vi "RemoteVI Hover Decision.vi"(0 "menus":T2(array[cluster]), 5 "state":T1, 7 "now":u32) -> (4 "navigate?":bool, 6 "dwell?":bool, 8 "parent?":bool, 10 "k":i32=-1)   [LabVIEW 2020, in "RemoteVI.lvlib"]
doc: "Decides what the remote pointer (state.x, state.y) asks of the open LabVIEW menus (RemoteVI List Menus.vi, deepest first): k is the menu under the pointer (RemoteVI Point On Popup.vi). navigate? - it is over the DEEPEST menu at a position not applied yet; dwell? - it has stayed on the highlighted item of the deepest menu (state.menu, state.hit) for 400 ms since row since and VK_RIGHT has not been posted for it; parent? - it is over a parent of open submenus at a position not applied yet. All three are FALSE when the pointer is over no menu, or when the deepest popup takes no keys (state.plain: colour picker, line width popup - neither it nor its parents can be driven with keys then). Pure."
uses:
  RemoteVI.lvlib
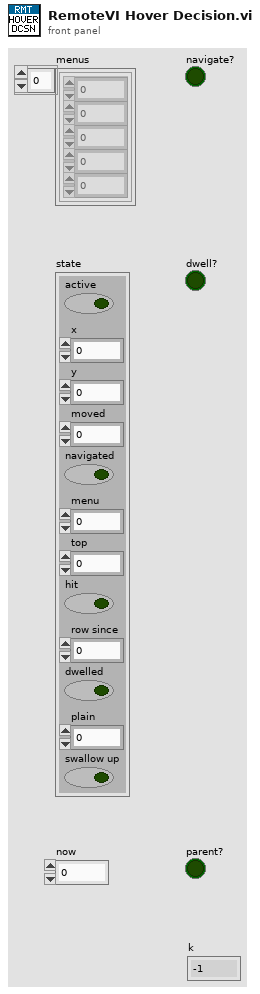
[diagram p1: front panel]
types:
  T1 = cluster{"active":bool, "x":i32, "y":i32, "moved":u32, "navigated":bool, "menu":u64, "top":i32, "hit":bool, "row since":u32, "dwelled":bool, "plain":u64, "swallow up":bool}
  T2 = cluster{"hwnd":u64, "x":i32, "y":i32, "w":i32, "h":i32}[]
  T3 = cluster{"hwnd":u64, "x":i32, "y":i32, "w":i32, "h":i32}
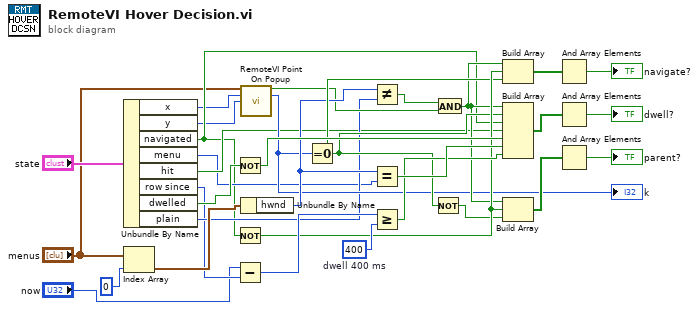
[diagram p0: block diagram]
diagram:
  w27 = u32 400  # dwell 400 ms
  n1 = Unbundle By Name("state") -> ("x"=w4:i32, "y"=w5:i32, "navigated"=w6:bool, "menu"=w7:u64, "hit"=w8:bool, "row since"=w9:u32, "dwelled"=w10:bool, "plain"=w11:u64)
  n2 = Index Array(array="menus", index=0) -> (element=w15:T3)
  n3 = Not(x=w10) -> (.not. x?=w30:bool)
  n4 = Not(x=w6) -> (.not. x?=w21:bool)
  n5 = Subtract(x="now", y=w9) -> (x-y=w26:u32)
  n6 = call "RemoteVI Point On Popup.vi"("windows"="menus", "x"=w4, "y"=w5) -> ("on popup?"=w12:bool, "index"=w13:i32)  [unwired: 11 in]
  "k" <- w13
  n7 = Unbundle By Name(w15) -> ("hwnd"=w16:u64)
  n8 = Equal To 0?(x=w13) -> (x = 0?=w19:bool)
  n9 = Not Equal?(x=w16, y=w11) -> (x != y?=w17:bool)
  n10 = Equal?(x=w16, y=w7) -> (x = y?=w29:bool)
  n11 = Greater Or Equal?(x=w26, y=w27) -> (x >= y?=w28:bool)
  n12 = Not(x=w19) -> (.not. x?=w20:bool)
  n13 = And(x=w17, y=w12) -> (x .and. y?=w18:bool)
  n14 = Build Array(w18, w21, w19) -> (w22:bool[])
  n15 = Build Array(w18, w19, w6, w8, w30, w29, w28) -> (w31:bool[])
  n16 = Build Array(w18, w21, w20) -> (w24:bool[])
  n17 = And Array Elements(Boolean array=w22) -> (logical AND=→"navigate?":bool)
  n18 = And Array Elements(Boolean array=w31) -> (logical AND=→"dwell?":bool)
  n19 = And Array Elements(Boolean array=w24) -> (logical AND=→"parent?":bool)
